vi "LabVIEW.Service.Wait(ms).vi"(9 "milliseconds to wait (1000)":u32=1000, 11 "Error In (no error)":errorcluster) -> (7 "Error Out":errorcluster)   [LabVIEW 2019]
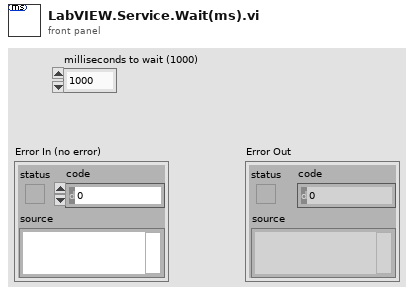
[diagram p1: front panel]
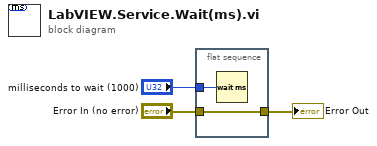
[diagram p0: block diagram]
diagram:
  n1 = flat-sequence {
    tunnel: [w5] -> w3
    tunnel: "Error In (no error)" -> [w5]
    tunnel: "milliseconds to wait (1000)" -> [w4]
    frame #0 {
      n2 = Wait (ms)(milliseconds to wait=w4) -> ()  [unwired: 1 out]
    }
  }
  "Error Out" <- w3
